vi "AlliGator Reset All Mouse Move Flags.vi"(8 "Error In":errorcluster) -> (0 "Error Out":errorcluster)   [LabVIEW 2021, in "AlliGator GUI.lvlib"]
uses:
  AlliGator GUI.lvlib
  Source Image/AlliGator Dataset Ctrl Refnums.ctl
  Phasor Plot/AlliGator Phasor Plot Ctrl Refnums.ctl
  Decay Fit Parameter Map/AlliGator Decay Fit Parameter Map Control Refnums.ctl
  Parameter Map/AlliGator Parameter Map Control Refnums.ctl
  Globals, Variables, Constants/AlliGator Refnums List.ctl
  Utilities/Read-Write.ctl
  Phasor Plot/AlliGator Phasor Plot.lvlib
  Decay Fit Parameter Map/AlliGator Decay Fit Parameter Map.lvlib
  Parameter Map/AlliGator Parameter Map.lvlib
  Utilities/Utilities.lvlib
panel:
  # "see the License on the block diagram (Ctrl+E or Window:Show Block Diagram)"
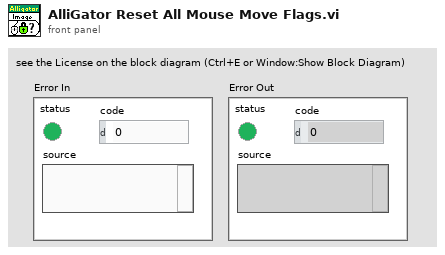
[diagram p1: front panel]
types:
  T1 = typedef "AlliGator GUI.lvlib/AlliGator Refnums List.ctl" = enum16{"---------- AlliGator Control Refnums ----------", "AlliGator Tab Control Refnum", "Dataset Ctrl Refnums", "Image Histogram Ctrl Refnums", "Intensity Time Trace Ctrl Refnums", "Decay Graph Ctrl Refnums", "Decay Statistics Graph Ctrl Refnums", "Phasor Graph Ctrl Refnums", "Phasor Ratio Graph Ctrl Refnums", "Phasor Plot Ctrl Refnums", "Lifetime & Other Parameters Ctrl Refnums", "Decay Fit Parameter Map Ctrl Refnums", "Parameter Map Ctrl Refnums", "Other AlliGator Ctrl Refnums", "---------- AlliGator Menu Refnums ----------", "AlliGator Menu", "---------- AlliGator VI Refnums ----------", "AlliGator Refnum", "AlliGator Settings Refnum", "AlliGator Launcher Refnum", "---------- IO Device ID ----------", "Mouse ID", "Keyboard ID"}
  T2 = typedef "AlliGator Parameter Map.lvlib/AlliGator Parameter Map Control Refnums.ctl" = cluster{"Parameter Map Color Scale":refnum<vi>, "Map Parameter":refnum<vi>, "Max Parameter":refnum<vi>, "Min Parameter":refnum<vi>, "Parameter Map Display":refnum<vi>, "Parameter Map Display Range":refnum<vi>, "Parameter Map Set":refnum<vi>, "Parameter Map X":refnum<vi>, "Parameter Map Y":refnum<vi>, "Parameter Map Value":refnum<vi>}
  T3 = typedef "AlliGator Decay Fit Parameter Map.lvlib/AlliGator Decay Fit Parameter Map Control Refnums.ctl" = cluster{"Decay Fit Parameter Map Color Scale":refnum<vi>, "Decay Fit Parameter":refnum<vi>, "Max Parameter":refnum<vi>, "Min Parameter":refnum<vi>, "Decay Fit Parameter Map Display":refnum<vi>, "Decay Fit Parameter Map Display Range":refnum<vi>, "Decay Parameter Map X":refnum<vi>, "Decay Parameter Map Y":refnum<vi>, "Decay Parameter Map Value":refnum<vi>}
  T4 = typedef "AlliGator Phasor Plot.lvlib/AlliGator Phasor Plot Ctrl Refnums.ctl" = cluster{"Phasor Ratio":refnum<vi>, "Modulus Lifetime":refnum<vi>, "Phasor at cursor (m, phi)":refnum<vi>, "Phase Lifetime":refnum<vi>, "Phasor at cursor (g, s)":refnum<vi>, "Phasor Plor Average Lifetime":refnum<vi>, "Phasor Plot Active":refnum<vi>, "Save Phasor Plot":refnum<vi>, "Image Overlay Color":refnum<vi>, "Phasor Plot Color Scale":refnum<vi>, "Reference 1 Button":refnum<vi>, "Reference 2 Button":refnum<vi>, "True Phasor Plot Value":refnum<vi>, "Phasor Plot Display Range":refnum<vi>, "Phasor Plot Display":refnum<vi>, "Phasor Plot Frequency":refnum<vi>, "Overlay Mode":refnum<vi>}
  T5 = typedef "AlliGator GUI.lvlib/AlliGator Dataset Ctrl Refnums.ctl" = cluster{"Current Data":refnum<vi>, "Gate Image Slide":refnum<vi>, "Time Point Slide":refnum<vi>, "Current Time Stamp":refnum<vi>, "Save Image":refnum<vi>, "Displayed Image":refnum<vi>, "Phasor Overlay Color":refnum<vi>, "Image Color Scale":refnum<vi>, "Use ROI as Search Area":refnum<vi>, "Source Image ROI Color":refnum<vi>, "True Pixel Value":refnum<vi>, "Source Image Display":refnum<vi>, "CPU":refnum<vi>}
  T6 = typedef "Utilities.lvlib/Read-Write.ctl" = enum16{"Read", "Write"}
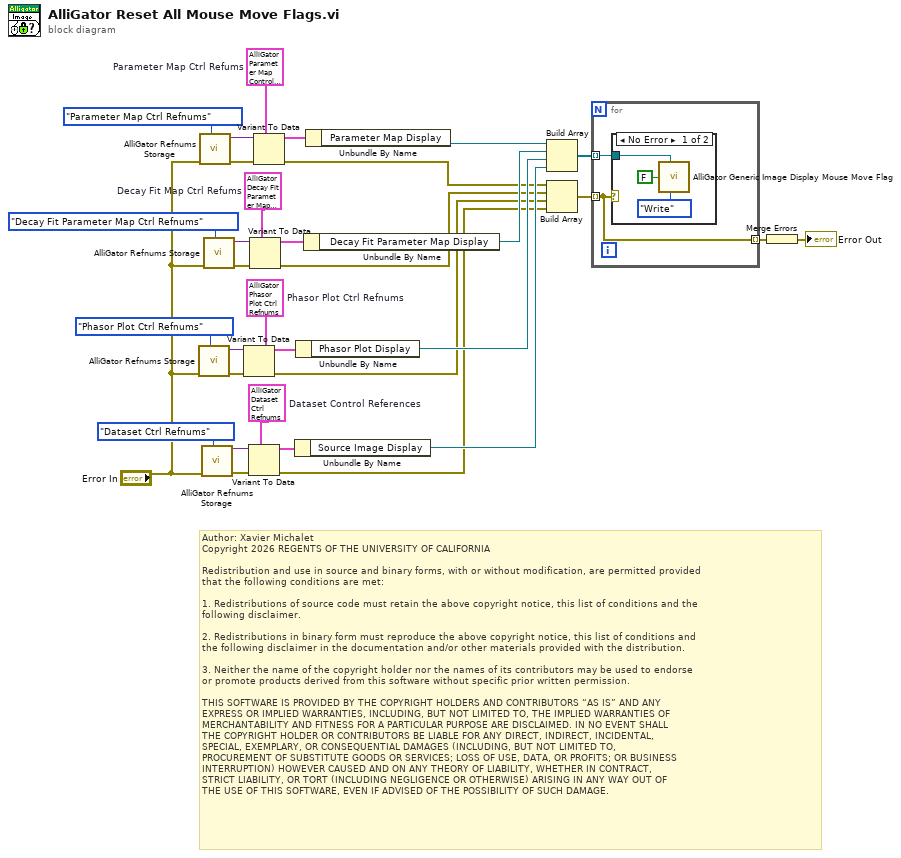
[diagram p0: block diagram]
diagram:
  w30 = T2 {"Parameter Map Color Scale"=refnum, "Map Parameter"=refnum, "Max Parameter"=refnum, "Min Parameter"=refnum, "Parameter Map Display"=refnum, "Parameter Map Display Range"=refnum, "Parameter Map Set"=refnum, "Parameter Map X"=refnum, "Parameter Map Y"=refnum, "Parameter Map Value"=refnum}  # Parameter Map Ctrl Refums
  w24 = T3 {"Decay Fit Parameter Map Color Scale"=refnum, "Decay Fit Parameter"=refnum, "Max Parameter"=refnum, "Min Parameter"=refnum, "Decay Fit Parameter Map Display"=refnum, "Decay Fit Parameter Map Display Range"=refnum, "Decay Parameter Map X"=refnum, "Decay Parameter Map Y"=refnum, "Decay Parameter Map Value"=refnum}  # Decay Fit Map Ctrl Refums
  w19 = T4 {"Phasor Ratio"=refnum, "Modulus Lifetime"=refnum, "Phasor at cursor (m, phi)"=refnum, "Phase Lifetime"=refnum, "Phasor at cursor (g, s)"=refnum, "Phasor Plor Average Lifetime"=refnum, "Phasor Plot Active"=refnum, "Save Phasor Plot"=refnum, "Image Overlay Color"=refnum, "Phasor Plot Color Scale"=refnum, "Reference 1 Button"=refnum, "Reference 2 Button"=refnum, "True Phasor Plot Value"=refnum, "Phasor Plot Display Range"=refnum, "Phasor Plot Display"=refnum, "Phasor Plot Frequency"=refnum, "Overlay Mode"=refnum}  # Phasor Plot Ctrl Refnums
  w14 = T5 {"Current Data"=refnum, "Gate Image Slide"=refnum, "Time Point Slide"=refnum, "Current Time Stamp"=refnum, "Save Image"=refnum, "Displayed Image"=refnum, "Phasor Overlay Color"=refnum, "Image Color Scale"=refnum, "Use ROI as Search Area"=refnum, "Source Image ROI Color"=refnum, "True Pixel Value"=refnum, "Source Image Display"=refnum, "CPU"=refnum}  # Dataset Control References
  # "Author: Xavier Michalet\nCopyright 2026 REGENTS OF THE UNIVERSITY OF CALIFORNIA\n\nRedistribution and use in source and binary forms, with or without modification, are permitted provided\nthat the following conditions are met:\n\n1. Redistributions of source code must retain the above copyright notice, this list of conditions and the\nfollowing disclaimer.\n\n2. Redistributions in binary form must reproduce the above copyright notice, this list of conditions and\nthe following disclaimer in the documentation and/or other materials provided with the distribution.\n\n3. Neither the name of the copyright holder nor the names of its contributors may be used to endorse \nor promote products derived from this software without specific prior written permission.\n\nTHIS SOFTWARE IS PROVIDED BY THE COPYRIGHT HOLDERS AND CONTRIBUTORS “AS IS” AND ANY \nEXPRESS OR IMPLIED WARRANTIES, INCLUDING, BUT NOT LIMITED TO, THE IMPLIED WARRANTIES OF\nMERCHANTABILITY AND FITNESS FOR A PARTICULAR PURPOSE ARE DISCLAIMED. IN NO EVENT SHALL\nTHE COPYRIGHT HOLDER OR CONTRIBUTORS BE LIABLE FOR ANY DIRECT, INDIRECT, INCIDENTAL, \nSPECIAL, EXEMPLARY, OR CONSEQUENTIAL DAMAGES (INCLUDING, BUT NOT LIMITED TO, \nPROCUREMENT OF SUBSTITUTE GOODS OR SERVICES; LOSS OF USE, DATA, OR PROFITS; OR BUSINESS\nINTERRUPTION) HOWEVER CAUSED AND ON ANY THEORY OF LIABILITY, WHETHER IN CONTRACT, \nSTRICT LIABILITY, OR TORT (INCLUDING NEGLIGENCE OR OTHERWISE) ARISING IN ANY WAY OUT OF\nTHE USE OF THIS SOFTWARE, EVEN IF ADVISED OF THE POSSIBILITY OF SUCH DAMAGE."
  n1 = call "AlliGator Refnums Storage.vi"("AlliGator Refnum List"=AlliGator_Refnums_List."Phasor Plot Ctrl Refnums", "Error In"="Error In") -> ("Error Out"=w20:errorcluster, "Data out"=w21:variant)  [unwired: 8 in]
  n2 = call "AlliGator Refnums Storage.vi"("AlliGator Refnum List"=AlliGator_Refnums_List."Parameter Map Ctrl Refnums", "Error In"="Error In") -> ("Error Out"=w31:errorcluster, "Data out"=w32:variant)  [unwired: 8 in]
  n3 = call "AlliGator Refnums Storage.vi"("AlliGator Refnum List"=AlliGator_Refnums_List."Dataset Ctrl Refnums", "Error In"="Error In") -> ("Error Out"=w16:errorcluster, "Data out"=w17:variant)  [unwired: 8 in]
  n4 = call "AlliGator Refnums Storage.vi"("AlliGator Refnum List"=AlliGator_Refnums_List."Decay Fit Parameter Map Ctrl Refnums", "Error In"="Error In") -> ("Error Out"=w26:errorcluster, "Data out"=w27:variant)  [unwired: 8 in]
  n5 = Variant To Data(error in=w20, type=w19, Variant=w21) -> (data=w22:T4, error out=w5:errorcluster)
  n6 = Variant To Data(error in=w16, type=w14, Variant=w17) -> (data=w18:T5, error out=w4:errorcluster)
  n7 = Variant To Data(error in=w26, type=w24, Variant=w27) -> (data=w28:T3, error out=w6:errorcluster)
  n8 = Variant To Data(error in=w31, type=w30, Variant=w32) -> (data=w29:T2, error out=w7:errorcluster)
  n9 = Unbundle By Name(w18) -> ("Source Image Display"=w9:refnum<vi>)
  n10 = Unbundle By Name(w22) -> ("Phasor Plot Display"=w10:refnum<vi>)
  n11 = Unbundle By Name(w28) -> ("Decay Fit Parameter Map Display"=w11:refnum<vi>)
  n12 = Unbundle By Name(w29) -> ("Parameter Map Display"=w12:refnum<vi>)
  n13 = Build Array(w12, w11, w10, w9) -> (w8:refnum<vi>[])
  n14 = Build Array(w7, w6, w5, w4) -> (w3:errorcluster[])
  n15 = for {
    tunnel: w8 -> [w35] mode=indexing
    tunnel: w3 -> [w34] mode=indexing
    tunnel: [w34] -> w2 mode=indexing
    n16 = case shown="No Error" w34 {
      tunnel: w35 -> [w38 _]
      frame No Error {
        n17 = call "AlliGator Generic Image Display Mouse Move Flag.vi"("Image Control Refnum"=w38, "Flag (in)"=FALSE, "Read/Write"=Read-Write."Write") -> ()  [unwired: 6 in, 1 out]
      }
      frame Error {
      }
    }
  }
  n18 = Merge Errors(w2) -> (→"Error Out":errorcluster)
